vi "Main.vi"(8 "error in (no error)":errorcluster caption="错误输入（无错误）") -> (0 "error out":errorcluster caption="错误输出")   [LabVIEW 2018]
doc: "该模板用于创建子VI。"
uses:
  D:/black&white/labview/Othello_Basic/bin/Othello.Basic.dll
  bin/Othello.Basic.dll
panel:
  in  "OthelloPanel":refnum<k24>(container)
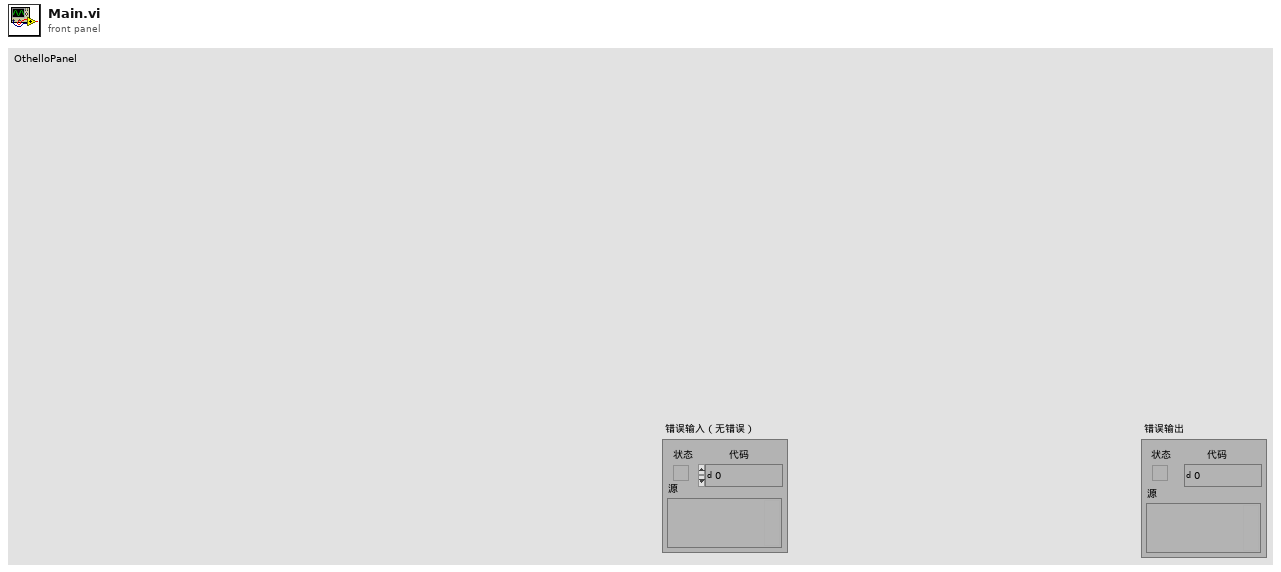
[diagram p1: front panel]
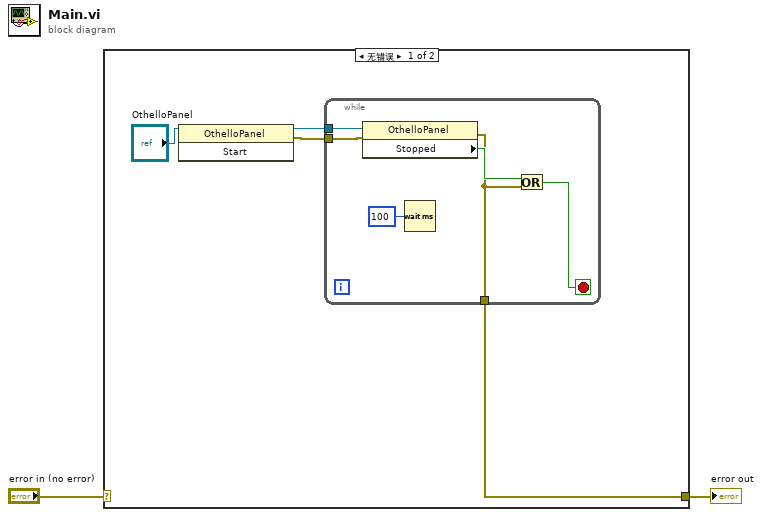
[diagram p0: block diagram]
diagram:
  n1 = case shown="无错误" "error in (no error)" {
    selector: "error in (no error)" -> [_ w13]
    tunnel: [w3 w13] -> w1
    frame No Error {
      n2 = invoke class="OthelloPanel" method="Start"(reference="OthelloPanel") -> (reference out=w5:refnum<k24>, error out=w4:errorcluster)  [unwired: 2 in, 1 out]
      n3 = while {
        tunnel: w5 -> [w12]
        tunnel: w4 -> [w11]
        tunnel: [w9] -> w3
        stop <- w8 stop-if-true
        n4 = property class="OthelloPanel"(reference=w12, error in=w11) -> (error out=w9:errorcluster, "Stopped"=w10:bool)  [unwired: 1 out]
        n5 = Wait (ms)(milliseconds to wait=u32 100 ("等待时间（毫秒）")) -> ()  [unwired: 1 out]
        n6 = Or(x=w10, y=w9) -> (x .or. y?=w8:bool)
      }
    }
    frame Error {
    }
  }
  "error out" <- w1
